vi "Regenerate Settings.vi"() -> (0 "Default Settings":T1)   [LabVIEW 2021, in "Settings.lvlib"]
doc: "Regenerate the default settings for the application and save to a new file.\n\nAlso copy the existing XML settings file to a .bak file."
uses:
  Settings.lvlib
  Settings.ctl
  Acquisition/Hardware Configuration.ctl
  Acquisition/Channel Settings.ctl
  Acquisition/IO Device.ctl
  Acquisition/Sensor Type.ctl
  Interval Timer/Repeat Interval.ctl
  Interval Timer/Interval Length.ctl
  Interval Timer/Interval Token.ctl
  Acquisition/IO Context.ctl
  Acquisition/IO API.ctl
  Logging/Logging Configuration.ctl
  Logging/Logging Mode.ctl
  Diagnostics/Diagnostics Configuration.ctl
  controls/Graph Settings.ctl
  Acquisition/Acquisition.lvlib
  Interval Timer/Interval Timer.lvlib
  Diagnostics/Diagnostics.lvlib
  Logging/Logging.lvlib
panel:
  out "(ignored) error out":errorcluster
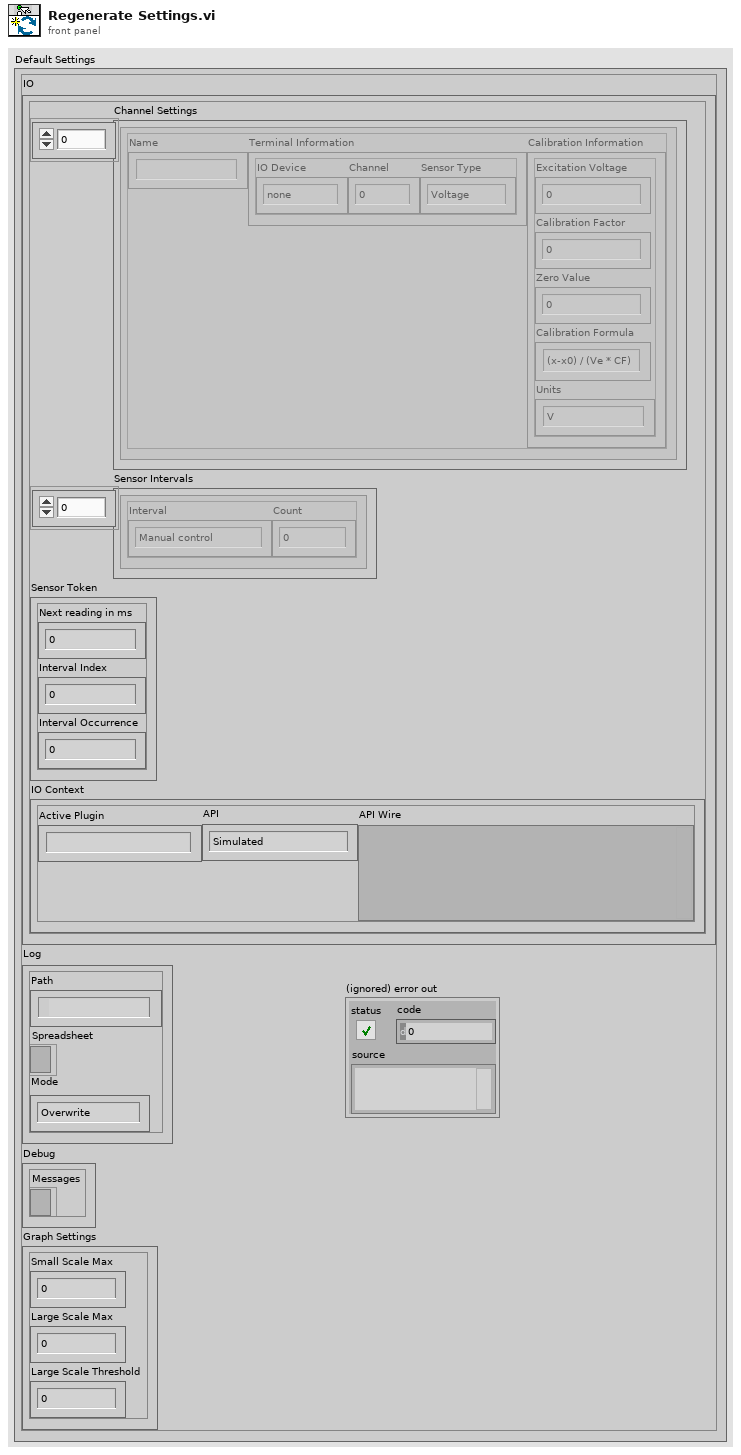
[diagram p1: front panel]
types:
  T1 = typedef "Settings.lvlib/Settings.ctl" = cluster{"IO":T2, "Log":T11, "Debug":T13, "Graph Settings":T14}
  T2 = typedef "Acquisition.lvlib/Hardware Configuration.ctl" = cluster{"Channel Settings":T3[], "Sensor Intervals":T6[], "Sensor Token":T8, "IO Context":T9}
  T3 = typedef "Acquisition.lvlib/Channel Settings.ctl" = cluster{"Name":string, "Terminal Information":cluster{"IO Device":T4, "Channel":i32, "Sensor Type":T5}, "Calibration Information":cluster{"Excitation Voltage":dbl, "Calibration Factor":dbl, "Zero Value":dbl, "Calibration Formula":string, "Units":string}}
  T4 = typedef "Acquisition.lvlib/IO Device.ctl" = enum16{"none", "9219", "9401"}
  T5 = typedef "Acquisition.lvlib/Sensor Type.ctl" = enum16{"Voltage", "Load", "Pressure", "Encoder"}
  T6 = typedef "Interval Timer.lvlib/Repeat Interval.ctl" = cluster{"Interval":T7, "Count":i32}
  T7 = typedef "Interval Timer.lvlib/Interval Length.ctl" = enum16{"Manual control", "1 second", "10 seconds", "30 seconds", "60 seconds", "600 seconds", "1200 seconds", "3600 seconds"}
  T8 = typedef "Interval Timer.lvlib/Interval Token.ctl" = cluster{"Next reading in ms":u32, "Interval Index":i32, "Interval Occurrence":i32}
  T9 = typedef "Acquisition.lvlib/IO Context.ctl" = cluster{"Active Plugin":string, "API":T10, "API Wire":variant}
  T10 = typedef "Acquisition.lvlib/IO API.ctl" = enum16{"Simulated", "DAQmx"}
  T11 = typedef "Logging.lvlib/Logging Configuration.ctl" = cluster{"Path":path, "Spreadsheet":refnum<file>, "Mode":T12}
  T12 = typedef "Logging.lvlib/Logging Mode.ctl" = enum16{"Overwrite", "Append", "Create New"}
  T13 = typedef "Diagnostics.lvlib/Diagnostics Configuration.ctl" = cluster{"Messages":refnum<file>}
  T14 = typedef "Graph Settings.ctl" = cluster{"Small Scale Max":dbl, "Large Scale Max":dbl, "Large Scale Threshold":dbl}
  T15 = cluster{"IO Device":T4, "Channel Number":i32, "Sensor Type":T5}
  T16 = cluster{"Excitation Voltage":dbl, "Calibration Factor":dbl, "Zero Value":dbl, "Calibration Formula":string, "Units":string}
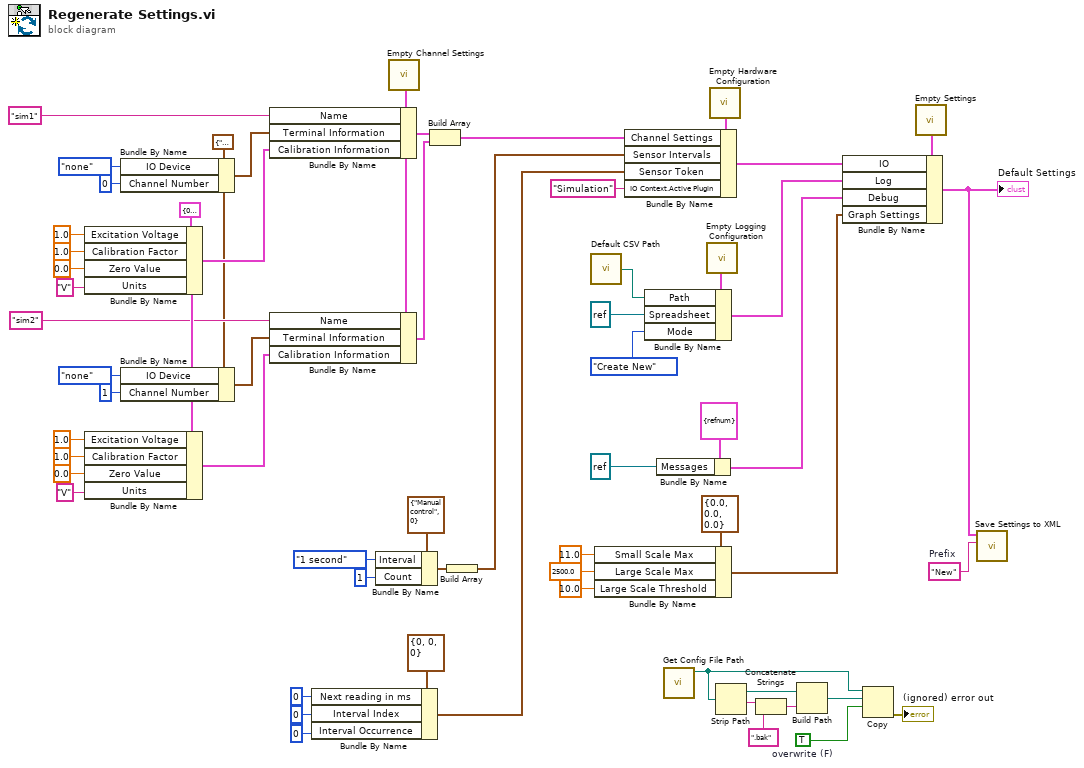
[diagram p0: block diagram]
diagram:
  w7 = T15 {"IO Device"=enum."none", "Channel Number"=0, "Sensor Type"=enum."Voltage"} ("Terminal Information")
  w15 = TRUE  # overwrite (F)
  w36 = T16 {"Excitation Voltage"=0.0, "Calibration Factor"=0.0, "Zero Value"=0.0, "Calibration Formula"="", "Units"=""} ("Calibration Information")
  w61 = "New"  # Prefix
  n1 = Bundle By Name(cluster=w36, "Excitation Voltage"=1.0, "Calibration Factor"=1.0, "Zero Value"=0.0, "Units"="V") -> (w35:T16)
  n2 = Bundle By Name(cluster=w36, "Excitation Voltage"=1.0, "Calibration Factor"=1.0, "Zero Value"=0.0, "Units"="V") -> (w34:T16)
  n3 = Bundle By Name(cluster=w7, "IO Device"=IO_Device."none", "Channel Number"=0) -> (w38:T15)
  n4 = Bundle By Name(cluster=w7, "IO Device"=IO_Device."none", "Channel Number"=1) -> (w37:T15)
  n5 = Bundle By Name(cluster=T8 {"Next reading in ms"=0, "Interval Index"=0, "Interval Occurrence"=0} ("Interval Token"), "Next reading in ms"=u32 0, "Interval Index"=0, "Interval Occurrence"=0) -> (w52:T8)
  n6 = Bundle By Name(cluster=T6 {"Interval"=enum."Manual control", "Count"=0} ("Repeat Interval"), "Interval"=Interval_Length."1 second", "Count"=1) -> (w51:T6)
  n7 = call "Empty Channel Settings.vi"() -> ("Channel Settings"=w14:T3)
  n8 = Bundle By Name(cluster=w14, "Name"="sim1", "Terminal Information"=w38, "Calibration Information"=w35) -> (w48:T3)
  n9 = Bundle By Name(cluster=w14, "Name"="sim2", "Terminal Information"=w37, "Calibration Information"=w34) -> (w39:T3)
  n10 = Build Array(w48, w39) -> (w49:T3[])
  n11 = Build Array(w51) -> (w50:T6[])
  n12 = call "Default CSV Path.vi"() -> ("CSV file path"=w47:path)
  n13 = Bundle By Name(cluster=T14 {"Small Scale Max"=0.0, "Large Scale Max"=0.0, "Large Scale Threshold"=0.0} ("Graph Settings"), "Small Scale Max"=11.0, "Large Scale Max"=2500.0, "Large Scale Threshold"=10.0) -> (w5:T14)
  n14 = Bundle By Name(cluster=T13 {"Messages"=refnum} ("Debug"), "Messages"=refnum<file> refnum) -> (w55:T13)
  n15 = call "Get Config File Path.vi"() -> ("XML File Path"=w17:path)  [unwired: 10 in, 1 out]
  n16 = call "Empty Logging Configuration.vi"() -> ("Logging Configuration"=w11:T11)
  n17 = Bundle By Name(cluster=w11, "Path"=w47, "Spreadsheet"=refnum<file> refnum, "Mode"=Logging_Mode."Create New") -> (w54:T11)
  n18 = call "Empty Hardware Configuration.vi"() -> ("Hardware Configuration"=w13:T2)
  n19 = Bundle By Name(cluster=w13, "Channel Settings"=w49, "Sensor Intervals"=w50, "Sensor Token"=w52, "IO Context.Active Plugin"="Simulation") -> (w53:T2)
  n20 = Strip Path(path=w17) -> (stripped path=w21:path, name=w20:string)
  n21 = Concatenate Strings(w20, ".bak" ("string")) -> (w18:string)
  n22 = Build Path(base path=w21, name or relative path=w18) -> (appended path=w16:path)
  n23 = Copy(9:w15, 10:w16, 11:w17) -> (0:→"(ignored) error out":errorcluster)  [unwired: 2 in, 2 out]
  n24 = call "Empty Settings.vi"() -> ("Settings"=w60:T1)
  n25 = Bundle By Name(cluster=w60, "IO"=w53, "Log"=w54, "Debug"=w55, "Graph Settings"=w5) -> (w59:T1)
  "Default Settings" <- w59
  n26 = call "Save Settings to XML.vi"("Prefix"=w61, "Settings"=w59) -> ()  [unwired: 9 in, 1 out]
